vi "set CHP Integration BW.vi"(8 "error in (no error)":errorcluster, 10 "Integration BW (Hz)":dbl, 11 "Keysight 9020A in":refnum<class "Keysight 9020A.lvclass">) -> (0 "error out":errorcluster, 3 "Keysight 9020A out":refnum<class "Keysight 9020A.lvclass">)   [LabVIEW 2023, in "Spectrum Analyzer.lvlib" / "Keysight 9020A.lvclass"]
uses:
  Keysight 9020A.lvclass
  Keysight 9020A.lvclass/Keysight 9020A.ctl
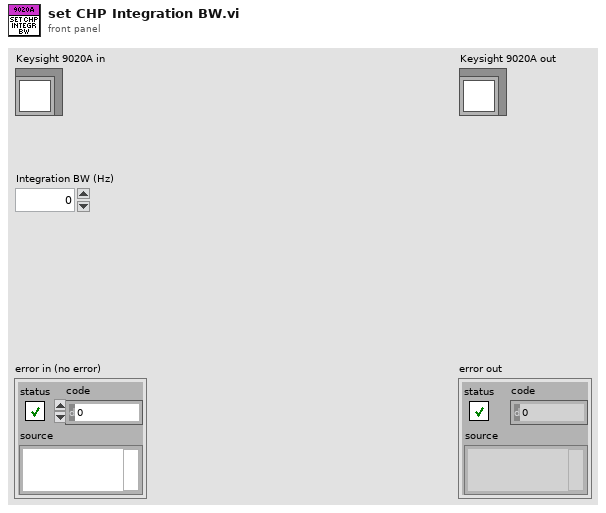
[diagram p1: front panel]
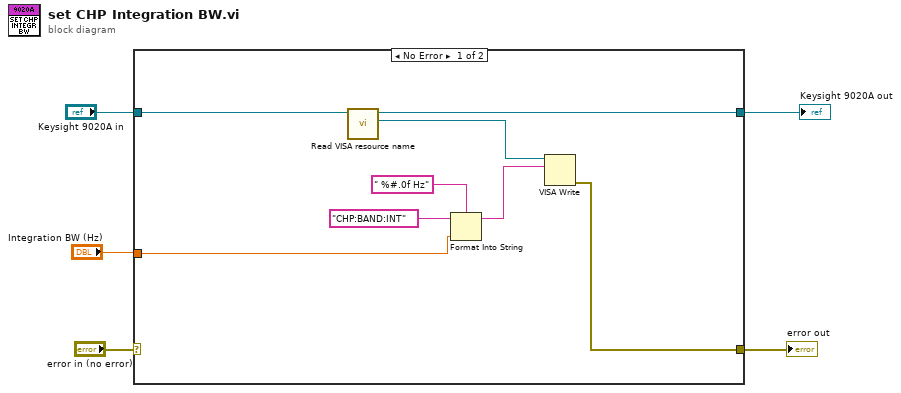
[diagram p0: block diagram]
diagram:
  n1 = case shown="No Error" "error in (no error)" {
    selector: "error in (no error)" -> [_ w14]
    tunnel: "Keysight 9020A in" -> [w8 w15]
    tunnel: [w13 w15] -> w4
    tunnel: [w10 w14] -> w2
    tunnel: "Integration BW (Hz)" -> [w9 _]
    frame No Error {
      n2 = call "Read VISA resource name.vi"("Keysight 9020A in"=w8) -> ("VISA resource name"=w12:refnum<visa-resource-name>, "Keysight 9020A out"=w13:refnum<class "Keysight 9020A.lvclass">)  [unwired: 8 in, 1 out]
      n3 = Format Into String(format string=" %#.0f Hz", initial string="CHP:BAND:INT", w9) -> (resulting string=w11:string)  [unwired: 1 in, 1 out]
      n4 = VISA Write(VISA resource name=w12, write buffer=w11) -> (error out=w10:errorcluster)  [unwired: 1 in, 2 out]
    }
    frame Error {
    }
  }
  "error out" <- w2
  "Keysight 9020A out" <- w4
